vi "Exo_factorielle_boucle.vi"(11 "N":i32) -> (0 "resultat du facto":i32)   [LabVIEW 2012]
panel:
  in  "N 2":i32
  out "FAC":i32
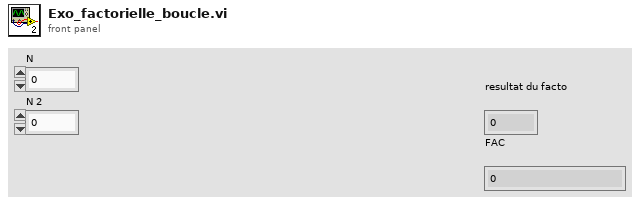
[diagram p1: front panel]
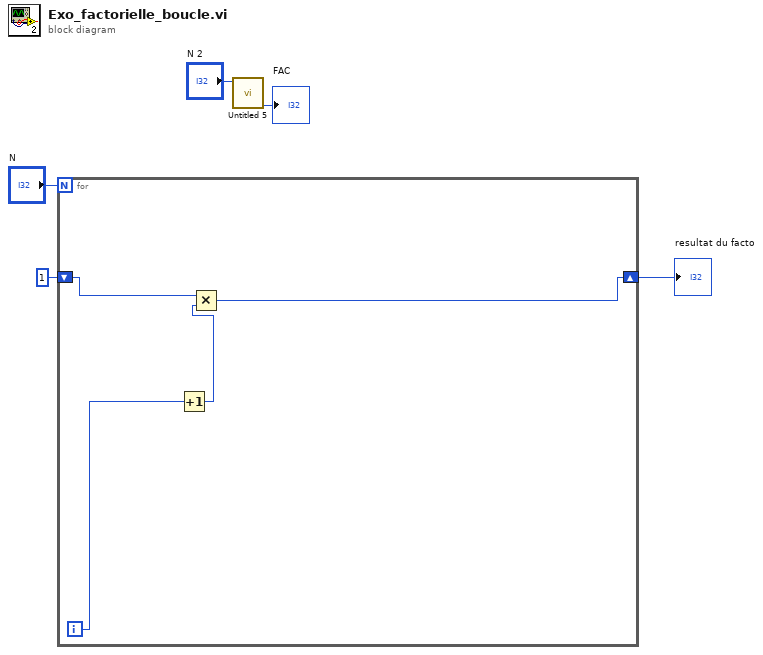
[diagram p0: block diagram]
diagram:
  n1 = for {
    N: "N" -> [_]
    shift-right: [w6] -> w4
    shift-left: 1 -> [w9]
    i -> [w8]
    n2 = Increment(x=w8) -> (x+1=w7:i32)
    n3 = Multiply(x=w9, y=w7) -> (x*y=w6:i32)
  }
  "resultat du facto" <- w4
  n4 = call "Untitled 5.vi"("N"="N 2") -> ("FAC"=→"FAC":i32)  [unwired: 10 in]
